vi "student_error_detect finish.vi"(4 "error in (no error)":errorcluster, 6 "key bit sequence":u8[](array[numeric]), 7 "input bit sequence":u8[](array[numeric])) -> (0 "error out":errorcluster, 3 "bit-error rate":dbl)   [LabVIEW 2022 SP3]
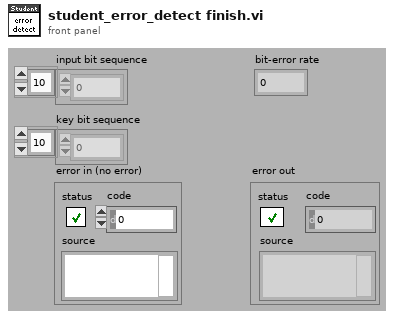
[diagram p1: front panel]
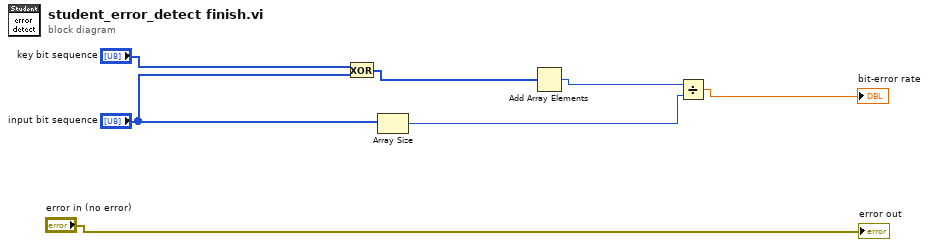
[diagram p0: block diagram]
diagram:
  n1 = Exclusive Or(1:"input bit sequence", 2:"key bit sequence") -> (0:w1:u8[])
  n2 = Array Size(array="input bit sequence") -> (size(s)=w4:i32)
  n3 = Add Array Elements(numeric array=w1) -> (sum=w6:u8)
  n4 = Divide(x=w6, y=w4) -> (x/y=→"bit-error rate":dbl)
  "error out" <- "error in (no error)"
